vi "Check PWM Pin.vi"(8 "error in (no error)":errorcluster, 11 "RPi PWM Pin in":T1) -> (0 "error out":errorcluster, 3 "RPi PWM Pin out":T1)   [LabVIEW 2020, in "wiringPi.lvlib"]
uses:
  wiringPi.lvlib
  <vilib>/ErrorRing/Error Ring.xnode
  <vilib>/Utility/error.llb/Error Cluster From Error Code.vi
  Type Defs/GPIO Pins.ctl
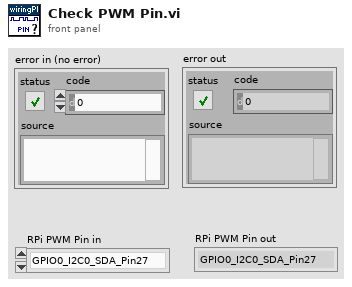
[diagram p1: front panel]
types:
  T1 = typedef "wiringPi.lvlib/GPIO Pins.ctl" = enum32{"GPIO0_I2C0_SDA_Pin27", "GPIO1_I2C0_SDA1_Pin28", "GPIO2_I2C1_SDA_Pin3", "GPIO3_I2C1_SCL_Pin5", "GPIO4_GPCLK0_Pin7", "GPIO5_GPCLK1_Pin29", "GPIO6_GPCLK2_Pin31", "GPIO7_SPI_CE1_N_Pin26", "GPIO8_SPI_CE0_N_Pin24", "GPIO9_SPI0_MISO_Pin21", "GPIO10_SPI0_MOSI_Pin19", "GPIO11_SPI0_CLK_Pin23", "GPIO12_PWM0_Pin32", "GPIO13_PWM1_Pin33", "GPIO14_TXD0_Pin8", "GPIO15_RXD0_Pin10", "GPIO16_Pin36", "GPIO17_Pin11", "GPIO18_PWM0_Pin12", "GPIO19_PWM1_Pin35", "GPIO20_GPCLK0_Pin38", "GPIO21_GPCLK1_Pin40", "GPIO22_Pin15", "GPIO23_Pin16", "GPIO24_Pin18", "GPIO25_Pin22", "GPIO26_Pin37", "GPIO27_Pin13"}
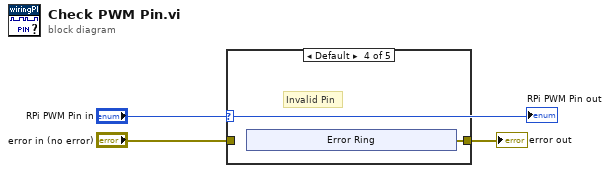
[diagram p0: block diagram]
diagram:
  n1 = case shown="Default" "RPi PWM Pin in" {
    tunnel: "error in (no error)" -> [w4 w5 w6 _ w13]
    tunnel: [w4 w5 w6 w7 w13] -> w1
    frame "GPIO12_PWM0_Pin32" {
    }
    frame "GPIO13_PWM1_Pin33" {
    }
    frame "GPIO18_PWM0_Pin12" {
    }
    frame Default {
      # "Invalid Pin"
      n2 = xnode "Error Ring"() -> ("error out"=w7:errorcluster)
    }
    frame "GPIO19_PWM1_Pin35" {
    }
  }
  "error out" <- w1
  "RPi PWM Pin out" <- "RPi PWM Pin in"
